vi "Initialize Scalar Datatype Classes.vi"(8 "error in (no error)":errorcluster, 9 "session in":u32, 10 "Register":T4={"Name"="", "Data Type"=enum."<Null>", "Default Value"=variant(dbl 0.0), "Attributes"=variant} {"Data Type" format="%.0x"}) -> (0 "error out":errorcluster, 2 "Register":T1={"Name"="", "Data Type"=enum."<Null>", "session"=0, "Scalar Type"=enum."Standard", "Index"=0, "Length"=0, "attributes"=variant(refnum<k20> refnum), "default value"=variant(refnum<k20> refnum)} {"Data Type" format="%.0x"})   [LabVIEW 2020, in "FPGA Addon Engine.lvlib"]
uses:
  FPGA Addon Engine.lvlib
  Addon Shared/Types/Register Information.ctl
  Addon Shared/Types/FPGA Addon Data Type.ctl
  Types/Register Settings.ctl
  Addon Shared/Types/Scalar Type.ctl
  Addon Shared/FPGA Addon Shared.lvlib
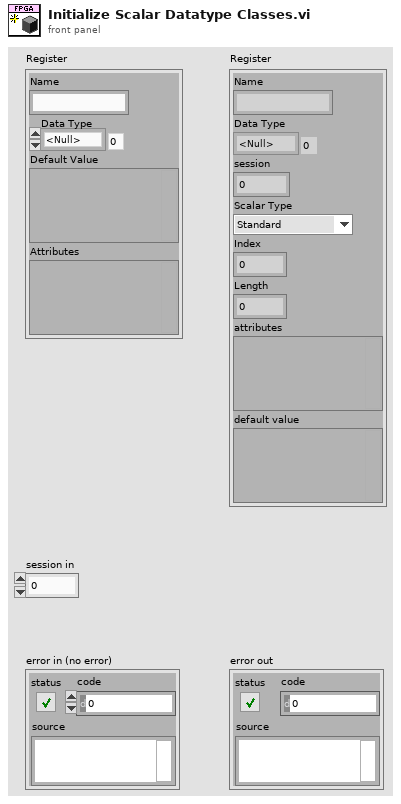
[diagram p1: front panel]
types:
  T1 = typedef "FPGA Addon Engine.lvlib/Register Settings.ctl" = cluster{"Name":string, "Data Type":T2, "session":u32, "Scalar Type":T3, "Index":i32, "Length":i32, "attributes":variant, "default value":variant}
  T2 = typedef "FPGA Addon Shared.lvlib/FPGA Addon Data Type.ctl" = enum8{"<Null>", "I8", "I16", "I32", "I64", "U8", "U16", "U32", "U64", "SGL", "Boolean", "Analog PWM In Settings", "Analog PWM In", "Digital PWM In Settings", "Digital PWM In", "Digital PWM Out", "Sine Out", "FXP", "FXP+/-24.5", "FXP+/-16.5", "FXP+/-32.8", "FXP+/-64.32", "FXP+/-16.7", "FXP+/-20.5", "FXP+/-27.5", "FXP+/-32.16", "FXP+16.3", "FXP+18.3", "Digital Static In", "Digital Static Out", "Digital Static In Settings", "Digital WSS Out", "Quad Encoder Settings", "Quad Encoder In", "Group"}
  T3 = typedef "FPGA Addon Shared.lvlib/Scalar Type.ctl" = enum16{"Standard", "Bitpacked"}
  T4 = typedef "FPGA Addon Shared.lvlib/Register Information.ctl" = cluster{"Name":string, "Data Type":T2, "Default Value":variant, "Attributes":variant}
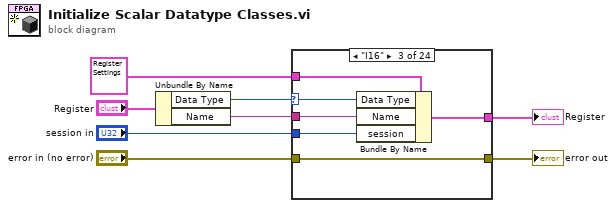
[diagram p0: block diagram]
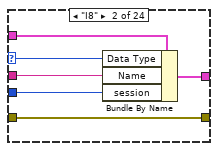
[diagram p3: hidden frame]
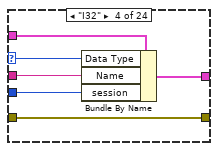
[diagram p4: hidden frame]
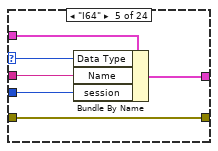
[diagram p5: hidden frame]
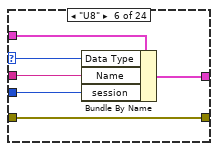
[diagram p6: hidden frame]
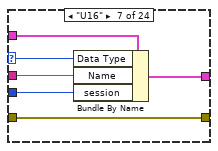
[diagram p7: hidden frame]
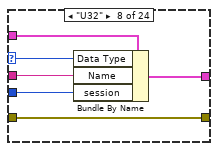
[diagram p8: hidden frame]
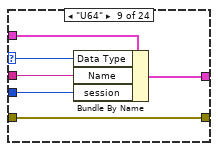
[diagram p9: hidden frame]
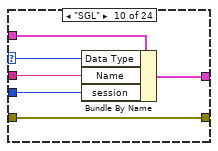
[diagram p10: hidden frame]
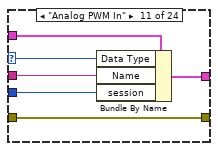
[diagram p11: hidden frame]
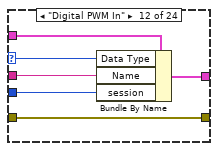
[diagram p12: hidden frame]
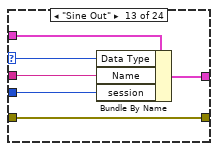
[diagram p13: hidden frame]
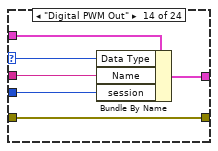
[diagram p14: hidden frame]
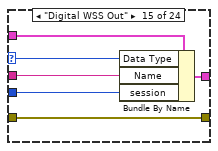
[diagram p15: hidden frame]
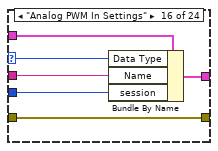
[diagram p16: hidden frame]
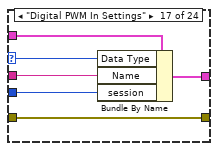
[diagram p17: hidden frame]
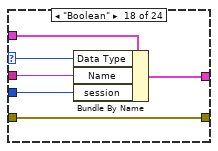
[diagram p18: hidden frame]
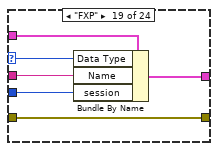
[diagram p19: hidden frame]
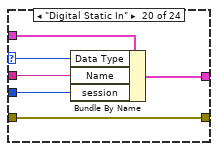
[diagram p20: hidden frame]
diagram:
  n1 = Unbundle By Name("Register") -> ("Data Type"=w3:T2, "Name"=w4:string)
  n2 = case shown="\"I16\"" w3 {
    selector: w3 -> [_ w16 w22 w28 w34 w40 w46 w52 w58 w64 w70 w76 w82 w88 w94 w100 w106 w112 w118 w124 w130 w136 w142 w148]
    tunnel: T1 {"Name"="", "Data Type"=enum."<Null>", "session"=0, "Scalar Type"=enum."Standard", "Index"=0, "Length"=0, "attributes"=variant(refnum<k20> refnum), "default value"=variant(refnum<k20> refnum)} ("Cluster") -> [w9 w13 w19 w25 w31 w37 w43 w49 w55 w61 w67 w74 w80 w85 w91 w97 w103 w109 w115 w121 w128 w133 w139 w146]
    tunnel: [w9 w15 w21 w27 w33 w39 w45 w51 w57 w63 w69 w75 w81 w87 w93 w99 w105 w111 w117 w123 w129 w135 w141 w147] -> w7
    tunnel: "error in (no error)" -> [w10 w14 w20 w26 w32 w38 w44 w50 w56 w62 w68 w73 w79 w86 w92 w98 w104 w110 w116 w122 w127 w134 w140 w145]
    tunnel: [w10 w14 w20 w26 w32 w38 w44 w50 w56 w62 w68 w73 w79 w86 w92 w98 w104 w110 w116 w122 w127 w134 w140 w145] -> w1
    tunnel: w4 -> [_ w12 w18 w24 w30 w36 w42 w48 w54 w60 w66 w72 w78 w84 w90 w96 w102 w108 w114 w120 w126 w131 w138 w144]
    tunnel: "session in" -> [_ w11 w17 w23 w29 w35 w41 w47 w53 w59 w65 w71 w77 w83 w89 w95 w101 w107 w113 w119 w125 w132 w137 w143]
    frame "<Null>", Default {
    }
    frame "I8" {
      n3 = Bundle By Name(cluster=w13, "Data Type"=w16, "Name"=w12, "session"=w11) -> (w15:T1)
    }
    frame "I16" {
      n4 = Bundle By Name(cluster=w19, "Data Type"=w22, "Name"=w18, "session"=w17) -> (w21:T1)
    }
    frame "I32" {
      n5 = Bundle By Name(cluster=w25, "Data Type"=w28, "Name"=w24, "session"=w23) -> (w27:T1)
    }
    frame "I64" {
      n6 = Bundle By Name(cluster=w31, "Data Type"=w34, "Name"=w30, "session"=w29) -> (w33:T1)
    }
    frame "U8" {
      n7 = Bundle By Name(cluster=w37, "Data Type"=w40, "Name"=w36, "session"=w35) -> (w39:T1)
    }
    frame "U16" {
      n8 = Bundle By Name(cluster=w43, "Data Type"=w46, "Name"=w42, "session"=w41) -> (w45:T1)
    }
    frame "U32" {
      n9 = Bundle By Name(cluster=w49, "Data Type"=w52, "Name"=w48, "session"=w47) -> (w51:T1)
    }
    frame "U64" {
      n10 = Bundle By Name(cluster=w55, "Data Type"=w58, "Name"=w54, "session"=w53) -> (w57:T1)
    }
    frame "SGL" {
      n11 = Bundle By Name(cluster=w61, "Data Type"=w64, "Name"=w60, "session"=w59) -> (w63:T1)
    }
    frame "Analog PWM In" {
      n12 = Bundle By Name(cluster=w67, "Data Type"=w70, "Name"=w66, "session"=w65) -> (w69:T1)
    }
    frame "Digital PWM In" {
      n13 = Bundle By Name(cluster=w74, "Data Type"=w76, "Name"=w72, "session"=w71) -> (w75:T1)
    }
    frame "Sine Out" {
      n14 = Bundle By Name(cluster=w80, "Data Type"=w82, "Name"=w78, "session"=w77) -> (w81:T1)
    }
    frame "Digital PWM Out" {
      n15 = Bundle By Name(cluster=w85, "Data Type"=w88, "Name"=w84, "session"=w83) -> (w87:T1)
    }
    frame "Digital WSS Out" {
      n16 = Bundle By Name(cluster=w91, "Data Type"=w94, "Name"=w90, "session"=w89) -> (w93:T1)
    }
    frame "Analog PWM In Settings" {
      n17 = Bundle By Name(cluster=w97, "Data Type"=w100, "Name"=w96, "session"=w95) -> (w99:T1)
    }
    frame "Digital PWM In Settings" {
      n18 = Bundle By Name(cluster=w103, "Data Type"=w106, "Name"=w102, "session"=w101) -> (w105:T1)
    }
    frame "Boolean" {
      n19 = Bundle By Name(cluster=w109, "Data Type"=w112, "Name"=w108, "session"=w107) -> (w111:T1)
    }
    frame "FXP" {
      n20 = Bundle By Name(cluster=w115, "Data Type"=w118, "Name"=w114, "session"=w113) -> (w117:T1)
    }
    frame "Digital Static In" {
      n21 = Bundle By Name(cluster=w121, "Data Type"=w124, "Name"=w120, "session"=w119) -> (w123:T1)
    }
    frame "Digital Static Out" {
      n22 = Bundle By Name(cluster=w128, "Data Type"=w130, "Name"=w126, "session"=w125) -> (w129:T1)
    }
    frame "Quad Encoder Settings" {
      n23 = Bundle By Name(cluster=w133, "Data Type"=w136, "Name"=w131, "session"=w132) -> (w135:T1)
    }
    frame "Quad Encoder In" {
      n24 = Bundle By Name(cluster=w139, "Data Type"=w142, "Name"=w138, "session"=w137) -> (w141:T1)
    }
    frame "Digital Static In Settings" {
      n25 = Bundle By Name(cluster=w146, "Data Type"=w148, "Name"=w144, "session"=w143) -> (w147:T1)
    }
  }
  "Register" <- w7
  "error out" <- w1
